vi "wait on clock.vi"(8 "error in":errorcluster, 10 "dt":u32=1, 11 "timing source in":refnum<class "scan engine timing source.lvclass">) -> (0 "error out":errorcluster, 2 "ticks since last call":u32, 3 "timing source out":refnum<class "scan engine timing source.lvclass">)   [LabVIEW 2013, in "scan engine timing source.lvclass"]
doc: "This core timing function is used inside of a loop to wait for a clock signal, or dt ticks of a clock signal."
uses:
  scan engine timing source.lvclass
  scan engine timing source.lvclass/scan engine timing source.ctl
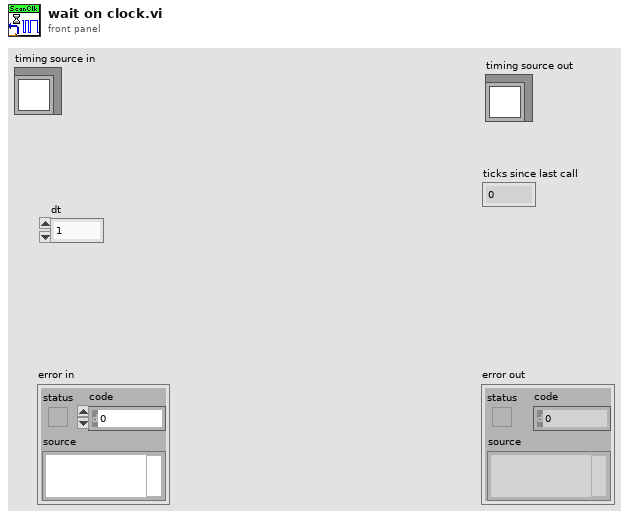
[diagram p1: front panel]
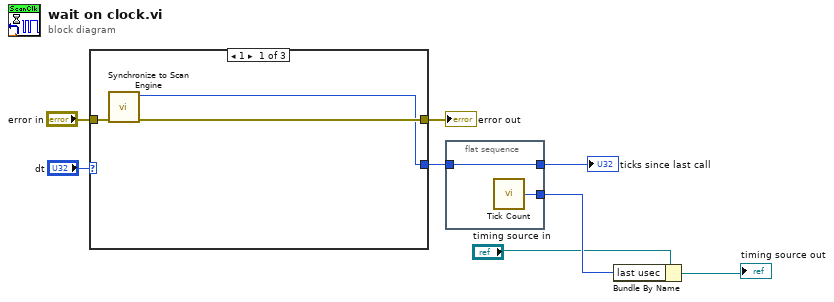
[diagram p0: block diagram]
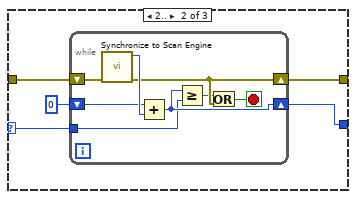
[diagram p2: hidden frame]
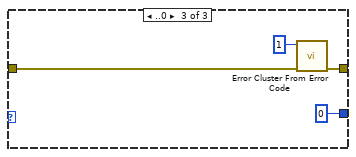
[diagram p3: hidden frame]
diagram:
  n1 = case shown="1" "dt" {
    selector: "dt" -> [_ w12 _]
    tunnel: "error in" -> [w11 w16 w28]
    tunnel: [w10 w15 w26] -> w7
    tunnel: [w9 w13 u32 0 ("scans since last call")] -> w5
    frame 1 {
      n2 = call <vilib>:"Synchronize to Scan Engine.vi"("error in (no error)"=w11) -> ("error out"=w10:errorcluster, "scans since last call"=w9:u32)  [unwired: 9 in]
    }
    frame 2.. {
      n3 = while {
        shift-right: [w20] -> w15
        shift-left: w16 -> [w24]
        shift-right: [w19] -> w13
        shift-left: u32 0 ("scans since last call") -> [w22]
        tunnel: w12 -> [w18]
        stop <- w21 stop-if-true
        n4 = call <vilib>:"Synchronize to Scan Engine.vi"("error in (no error)"=w24) -> ("error out"=w20:errorcluster, "scans since last call"=w23:u32)  [unwired: 9 in]
        n5 = Add(x=w22, y=w23) -> (x+y=w19:u32)
        n6 = Greater Or Equal?(x=w19, y=w18) -> (x >= y?=w17:bool)
        n7 = Or(x=w17, y=w20) -> (x .or. y?=w21:bool)
      }
    }
    frame ..0 {
      n8 = call <vilib>:"Error Cluster From Error Code.vi"("error in (no error)"=w28, "error code (0)"=1) -> ("error out"=w26:errorcluster)  [unwired: 7 in]
    }
  }
  "error out" <- w7
  n9 = flat-sequence {
    tunnel: w5 -> [w30]
    tunnel: [w30] -> w4
    tunnel: [w29] -> w3
    frame #0 {
      n10 = call "Tick Count"() -> ("Tick Count(uSec)"=w29:u32)
    }
  }
  n11 = Bundle By Name(cluster="timing source in", "last usec"=w3) -> (→"timing source out":refnum<class "scan engine timing source.lvclass">)
  "ticks since last call" <- w4
